vi "Read.vi"(8 "error in (no error)":errorcluster, 9 "bytes to read":i32, 10 "timeout us (-1)":i64=-1, 11 "pipe reader in":refnum<data-value>) -> (0 "error out":errorcluster, 1 "bytes read":i32, 2 "data":string, 3 "pipe reader out":refnum<data-value>, 4 "timed out?":bool)   [LabVIEW 2016, in "Linux RT IPC.Pipes.lvlib" / "Unix Pipe Reader.lvclass"]
doc: "This VI reads a certain number of bytes from the provided pipe endpoint."
uses:
  Unix Pipe Reader.lvclass
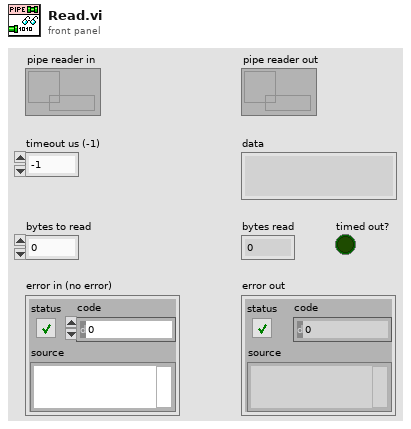
[diagram p1: front panel]
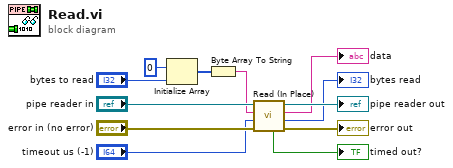
[diagram p0: block diagram]
diagram:
  n1 = Initialize Array(u8 0 ("element"), "bytes to read") -> (w6:u8[])
  n2 = Byte Array To String(unsigned byte array=w6) -> (string=w5:string)
  n3 = call "Read (In Place).vi"("error in (no error)"="error in (no error)", "timeout us (-1)"="timeout us (-1)", "preallocated data in"=w5, "pipe reader in"="pipe reader in") -> ("error out"=→"error out":errorcluster, "bytes read"=→"bytes read":i32, "data out"=→"data":string, "pipe reader out"=→"pipe reader out":refnum<data-value>, "timed out?"=→"timed out?":bool)  [unwired: 3 in]
